vi "Start Async.vi"(8 "error in (no error)":errorcluster, 11 "gRPC service in":refnum<class "ThermalChamberController.lvclass">) -> (0 "error out":errorcluster, 3 "gRPC service out":refnum<class "ThermalChamberController.lvclass">)   [LabVIEW 2020, in "thermal-chamber-controller_server.lvlib" / "ThermalChamberController.lvclass"]
uses:
  ThermalChamberController.lvclass
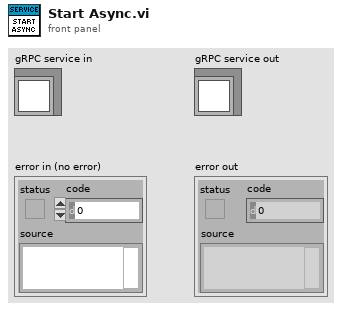
[diagram p1: front panel]
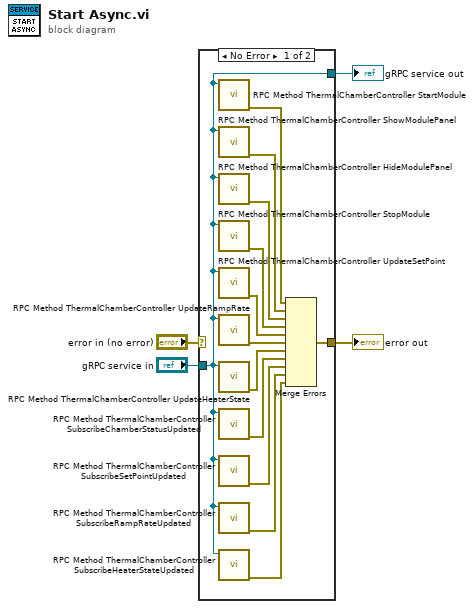
[diagram p0: block diagram]
diagram:
  n1 = case shown="No Error" "error in (no error)" {
    selector: "error in (no error)" -> [_ w19]
    tunnel: [w17 w19] -> w3
    tunnel: [w16 w18] -> w1
    tunnel: "gRPC service in" -> [w16 w18]
    frame No Error {
      n2 = call "RPC Method ThermalChamberController StartModule.vi"("gRPC service in"=w16) -> ("error out"=w15:errorcluster)  [unwired: 9 in, 1 out]
      n3 = call "RPC Method ThermalChamberController ShowModulePanel.vi"("gRPC service in"=w16) -> ("error out"=w14:errorcluster)  [unwired: 9 in, 1 out]
      n4 = call "RPC Method ThermalChamberController HideModulePanel.vi"("gRPC service in"=w16) -> ("error out"=w13:errorcluster)  [unwired: 9 in, 1 out]
      n5 = call "RPC Method ThermalChamberController StopModule.vi"("gRPC service in"=w16) -> ("error out"=w12:errorcluster)  [unwired: 9 in, 1 out]
      n6 = call "RPC Method ThermalChamberController UpdateSetPoint.vi"("gRPC service in"=w16) -> ("error out"=w11:errorcluster)  [unwired: 9 in, 1 out]
      n7 = call "RPC Method ThermalChamberController UpdateRampRate.vi"("gRPC service in"=w16) -> ("error out"=w10:errorcluster)  [unwired: 9 in, 1 out]
      n8 = call "RPC Method ThermalChamberController UpdateHeaterState.vi"("gRPC service in"=w16) -> ("error out"=w9:errorcluster)  [unwired: 9 in, 1 out]
      n9 = call "RPC Method ThermalChamberController SubscribeChamberStatusUpdated.vi"("gRPC service in"=w16) -> ("error out"=w8:errorcluster)  [unwired: 9 in, 1 out]
      n10 = call "RPC Method ThermalChamberController SubscribeSetPointUpdated.vi"("gRPC service in"=w16) -> ("error out"=w7:errorcluster)  [unwired: 9 in, 1 out]
      n11 = call "RPC Method ThermalChamberController SubscribeRampRateUpdated.vi"("gRPC service in"=w16) -> ("error out"=w6:errorcluster)  [unwired: 9 in, 1 out]
      n12 = call "RPC Method ThermalChamberController SubscribeHeaterStateUpdated.vi"("gRPC service in"=w16) -> ("error out"=w5:errorcluster)  [unwired: 9 in, 1 out]
      n13 = Merge Errors(w15, w14, w13, w12, w11, w10, w9, w8, w7, w6, w5) -> (w17:errorcluster)
    }
    frame Error {
    }
  }
  "error out" <- w3
  "gRPC service out" <- w1
